vi "Read Item Names.vi"(8 "error in (no error)":errorcluster, 11 "Selector in":refnum<class "Selector.lvclass">) -> (0 "error out":errorcluster, 2 "Item Names":string[][](array[string]), 3 "Selector out":refnum<class "Selector.lvclass">)   [LabVIEW 2019, in "Selector.lvclass"]
uses:
  Selector.lvclass
  Selector.lvclass/Selector.ctl
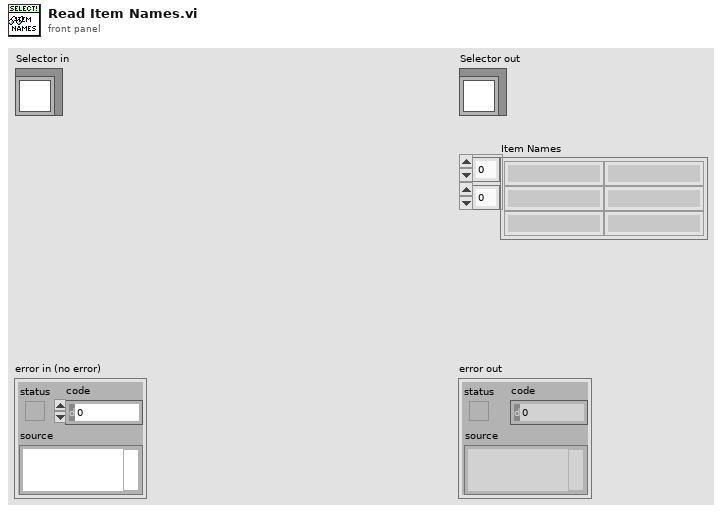
[diagram p1: front panel]
types:
  T1 = cluster{"Name":string, "Group":string, "Enabled":bool}[]
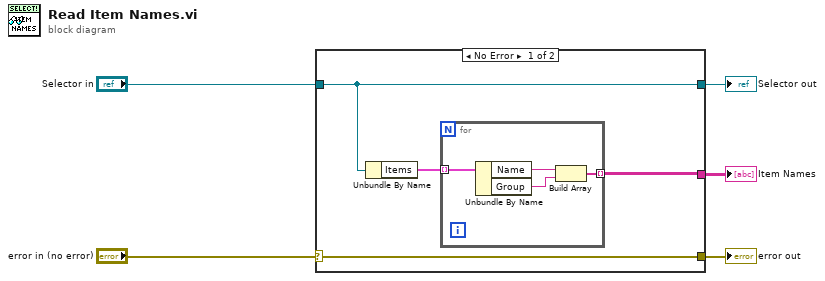
[diagram p0: block diagram]
diagram:
  n1 = case shown="No Error" "error in (no error)" {
    selector: "error in (no error)" -> [w9 w14]
    tunnel: [w9 w14] -> w4
    tunnel: [w8 w15] -> w3
    tunnel: "Selector in" -> [w8 w15]
    tunnel: [w6 _] -> w2
    frame No Error {
      n2 = Unbundle By Name(w8) -> ("Items"=w7:T1)
      n3 = for {
        tunnel: w7 -> [w13] mode=indexing
        tunnel: [w10] -> w6 mode=indexing
        n4 = Unbundle By Name(w13) -> ("Name"=w12:string, "Group"=w11:string)
        n5 = Build Array(w12, w11) -> (w10:string[])
      }
    }
    frame Error {
    }
  }
  "error out" <- w4
  "Selector out" <- w3
  "Item Names" <- w2
